vi "VIH Project - Get Effective File Rule - Abs Paths.vi"(10 "Build Root Dir":path, 11 "File Rule in":T1) -> (3 "File Rule out":T1)   [LabVIEW 2014]
doc: "::: VI Helpeks :::\nCopyright (c) 2000-2026 Konstantin Shifershteyn. All rights reserved."
uses:
  _VIH HelpGen.llb/VIH HelpGen Typedef - Cluster - File Rule.ctl
  _VIH HelpGen.llb/VIH HelpGen Typedef - Enum - Default,Enable,Disable.ctl
  _VIH HelpGen.llb/VIH HelpGen Typedef - Cluster - File Rule - Source Paths.ctl
  _VIH HelpGen.llb/VIH HelpGen Typedef - Cluster - File Rule - Target Paths.ctl
  _VIH HelpGen.llb/VIH HelpGen Typedef - Enum - Description Mode.ctl
  _VIH HelpGen.llb/VIH HelpGen Typedef - Cluster - Control Rule.ctl
  _VIH HelpGen.llb/VIH HelpGen Typedef - Cluster - Enum Value Info.ctl
  _VIH HelpGen.llb/VIH HelpGen Typedef - Cluster - Group Rule - Flags.ctl
panel:
  # "VI Helpeks\nCopyright (c) 2012-2026 Konstantin Shifershteyn"
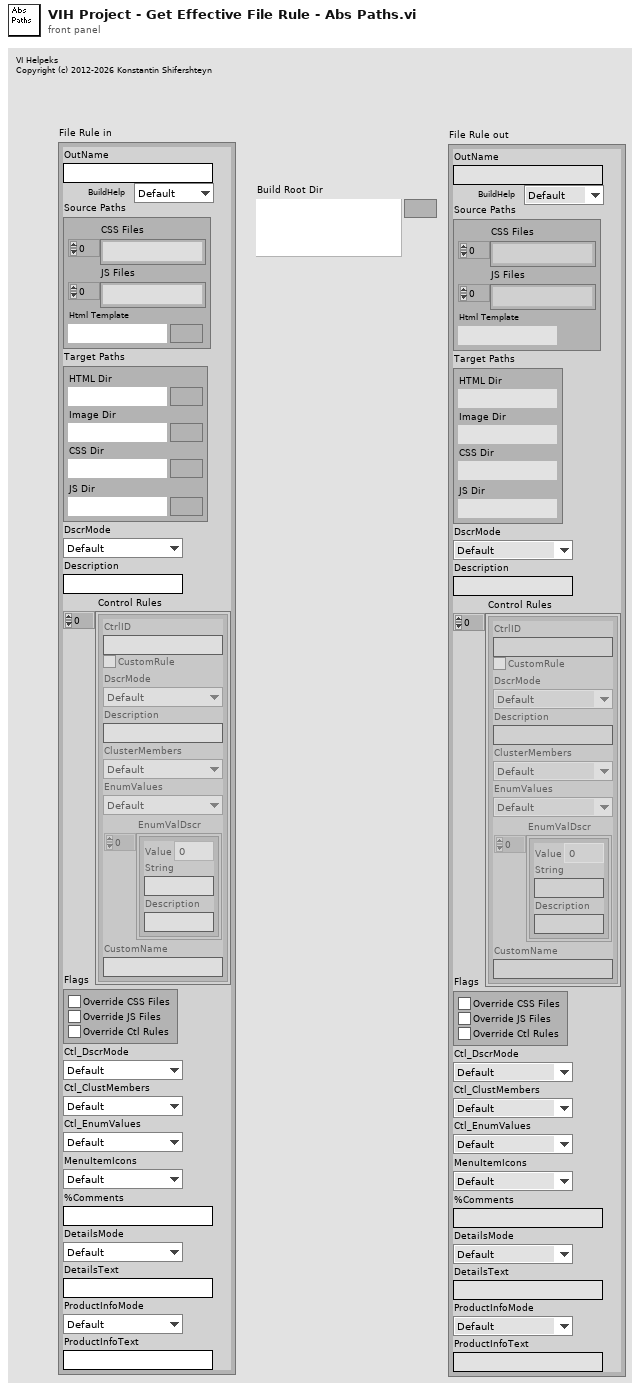
[diagram p1: front panel]
types:
  T1 = typedef "VIH HelpGen Typedef - Cluster - File Rule.ctl" = cluster{"OutName":string, "BuildHelp":T2, "Source Paths":T3, "Target Paths":T4, "DscrMode":T5, "Description":string, "Control Rules":T6[], "Flags":T8, "Ctl_DscrMode":T5, "Ctl_ClustMembers":T2, "Ctl_EnumValues":T2, "MenuItemIcons":T2, "%Comments":string, "DetailsMode":T5, "DetailsText":string, "ProductInfoMode":T2, "ProductInfoText":string}
  T2 = typedef "VIH HelpGen Typedef - Enum - Default,Enable,Disable.ctl" = enum16{"Default", "Enable", "Disable"}
  T3 = typedef "VIH HelpGen Typedef - Cluster - File Rule - Source Paths.ctl" = cluster{"CSS Files":path[], "JS Files":path[], "Html Template":path}
  T4 = typedef "VIH HelpGen Typedef - Cluster - File Rule - Target Paths.ctl" = cluster{"HTML Dir":path, "Image Dir":path, "CSS Dir":path, "JS Dir":path}
  T5 = typedef "VIH HelpGen Typedef - Enum - Description Mode.ctl" = enum16{"Default", "Description", "Description1", "Description2", "Custom", "None"}
  T6 = typedef "VIH HelpGen Typedef - Cluster - Control Rule.ctl" = cluster{"CtrlID":string, "CustomRule":bool, "DscrMode":T5, "Description":string, "ClusterMembers":T2, "EnumValues":T2, "EnumValDscr":T7[], "CustomName":string}
  T7 = typedef "VIH HelpGen Typedef - Cluster - Enum Value Info.ctl" = cluster{"Value":ext, "String":string, "Description":string}
  T8 = typedef "VIH HelpGen Typedef - Cluster - Group Rule - Flags.ctl" = cluster{"Override CSS Files":bool, "Override JS Files":bool, "Override Ctl Rules":bool}
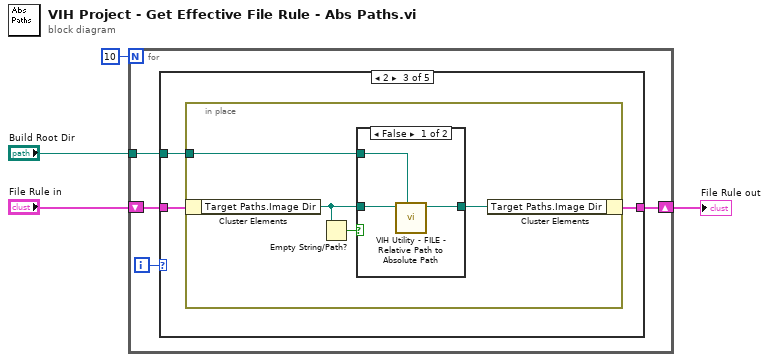
[diagram p0: block diagram]
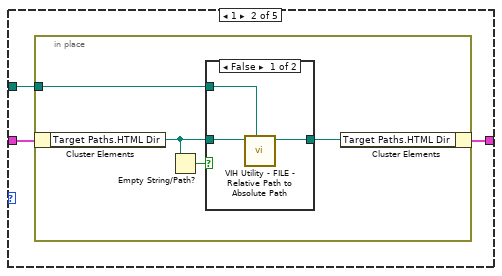
[diagram p3: hidden frame]
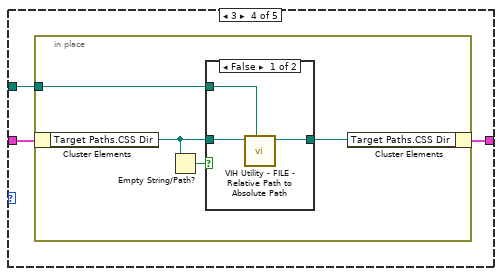
[diagram p6: hidden frame]
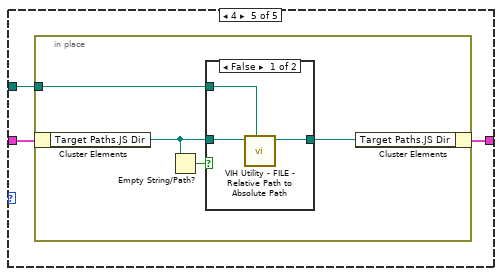
[diagram p8: hidden frame]
diagram:
  n1 = for {
    N: 10 -> [_]
    shift-right: [w5] -> w1
    shift-left: "File Rule in" -> [w8]
    tunnel: "Build Root Dir" -> [w7]
    i -> [w6]
    n2 = case shown="2" w6 {
      tunnel: w8 -> [w9 w12 w23 w34 w45]
      tunnel: w7 -> [_ w11 w22 w33 w44]
      tunnel: [w9 w10 w21 w32 w43] -> w5
      frame Default {
      }
      frame 1 {
        n3 = in-place {
          in-place-border: w11 -> [w15]
          n4 = in-place-cluster #1(w12) -> ("Target Paths.HTML Dir"=w13:path)
          n5 = Empty String/Path?(string/path=w13) -> (empty?=w14:bool)
          n6 = case shown="False" w14 {
            tunnel: w13 -> [w19 _]
            tunnel: [w18 w20] -> w16
            tunnel: w15 -> [w17 w20]
            frame False {
              n7 = call "VIH Utility - FILE - Relative Path to Absolute Path.vi"("base path (empty: dir of Top VI)"=w17, "Path"=w19) -> ("Path out"=w18:path)  [unwired: 8 in, 1 out]
            }
            frame True {
            }
          }
          n8 = in-place-cluster #1("Target Paths.HTML Dir"=w16) -> (w10:T1)
        }
      }
      frame 2 {
        n9 = in-place {
          in-place-border: w22 -> [w26]
          n10 = in-place-cluster #2(w23) -> ("Target Paths.Image Dir"=w24:path)
          n11 = Empty String/Path?(string/path=w24) -> (empty?=w25:bool)
          n12 = case shown="False" w25 {
            tunnel: w24 -> [w30 _]
            tunnel: [w29 w31] -> w27
            tunnel: w26 -> [w28 w31]
            frame False {
              n13 = call "VIH Utility - FILE - Relative Path to Absolute Path.vi"("base path (empty: dir of Top VI)"=w28, "Path"=w30) -> ("Path out"=w29:path)  [unwired: 8 in, 1 out]
            }
            frame True {
            }
          }
          n14 = in-place-cluster #2("Target Paths.Image Dir"=w27) -> (w21:T1)
        }
      }
      frame 3 {
        n15 = in-place {
          in-place-border: w33 -> [w37]
          n16 = in-place-cluster #3(w34) -> ("Target Paths.CSS Dir"=w35:path)
          n17 = Empty String/Path?(string/path=w35) -> (empty?=w36:bool)
          n18 = case shown="False" w36 {
            tunnel: w35 -> [w41 _]
            tunnel: [w40 w42] -> w38
            tunnel: w37 -> [w39 w42]
            frame False {
              n19 = call "VIH Utility - FILE - Relative Path to Absolute Path.vi"("base path (empty: dir of Top VI)"=w39, "Path"=w41) -> ("Path out"=w40:path)  [unwired: 8 in, 1 out]
            }
            frame True {
            }
          }
          n20 = in-place-cluster #3("Target Paths.CSS Dir"=w38) -> (w32:T1)
        }
      }
      frame 4 {
        n21 = in-place {
          in-place-border: w44 -> [w48]
          n22 = in-place-cluster #4(w45) -> ("Target Paths.JS Dir"=w46:path)
          n23 = Empty String/Path?(string/path=w46) -> (empty?=w47:bool)
          n24 = case shown="False" w47 {
            tunnel: w46 -> [w52 _]
            tunnel: [w51 w53] -> w49
            tunnel: w48 -> [w50 w53]
            frame False {
              n25 = call "VIH Utility - FILE - Relative Path to Absolute Path.vi"("base path (empty: dir of Top VI)"=w50, "Path"=w52) -> ("Path out"=w51:path)  [unwired: 8 in, 1 out]
            }
            frame True {
            }
          }
          n26 = in-place-cluster #4("Target Paths.JS Dir"=w49) -> (w43:T1)
        }
      }
    }
  }
  "File Rule out" <- w1
